vi "global.vi"() -> ()   [LabVIEW 2026, in "Core.lvlib"]
uses:
  Core.lvlib
panel:
  in  "Test Instruction":string
  in  "Iteration":u64
  in  "Frame Number":u32
  in  "Run ID Replay":string
  in  "Relative Seconds Frame 0":dbl format="%_19f"
  in  "Run ID":string
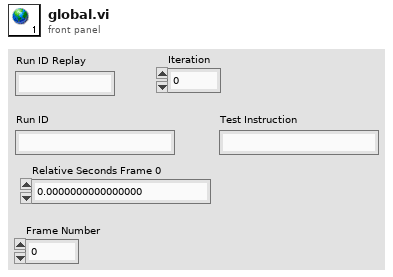
[diagram p1: front panel]
diagram:
